vi "Caller.vi"() -> ()   [LabVIEW 2020]
panel:
  out "Which Button?":T1(ring)=enum."Center Button"
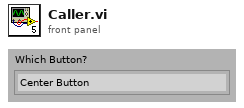
[diagram p1: front panel]
types:
  T1 = enum16{"Left Button", "Center Button", "Right Button", "Window Close"}
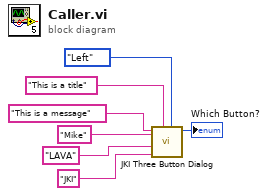
[diagram p0: block diagram]
diagram:
  n1 = call "JKI Three Button Dialog.vi"("Justify Message (Left)"=enum16{"Left", "Center", "Right"}."Left", "Window Title (\"\")"="This is a title" ("Window Title (\"\")"), "Right Button Text (\"Cancel\")"="JKI" ("Right Button Text (\"Cancel\")"), "Center Button Text (\"No\")"="LAVA" ("Center Button Text (\"No\")"), "Left Button Text (\"Yes\")"="Mike" ("Left Button Text (\"Yes\")"), "message"="This is a message") -> ("Which Button?"=→"Which Button?":T1)  [unwired: 5 in]
